vi "Engine_Tick.vi"(0 "Channels":T3, 5 "State":T1={"Tick"=0, "Phase"=0, "PhaseTicks"=0, "Level"=1, "Room"=0, "X10"=0, "Y10"=0, "VY10"=0, "Mode"=0, "Facing"=0, "Run"=0, "Vert"=0, "StandY"=0, "EntryX10"=0, "EntryY10"=0, "EntryMode"=0, "Lives"=4, "Score"=0, "NextLife"=10000, "KeyR"=0, "KeyB"=0, "KeyY"=0, "Torch"=FALSE, "FloorPhase"=0, "Dead"=FALSE, "LevelStart"=FALSE, "Quit"=FALSE, "Sound"=0, "Seed"=12345, "DemoStep"=0, "Tiles"=[], "World"=[], "Enemies"=[], "Highscores"=[], "Name"=[0, 0, 0], "Cursor"=0}, 7 "Rooms":T2(array[cluster]), 11 "error in":errorcluster) -> (4 "State out":T1={"Tick"=0, "Phase"=0, "PhaseTicks"=0, "Level"=1, "Room"=0, "X10"=0, "Y10"=0, "VY10"=0, "Mode"=0, "Facing"=0, "Run"=0, "Vert"=0, "StandY"=0, "EntryX10"=0, "EntryY10"=0, "EntryMode"=0, "Lives"=4, "Score"=0, "NextLife"=10000, "KeyR"=0, "KeyB"=0, "KeyY"=0, "Torch"=FALSE, "FloorPhase"=0, "Dead"=FALSE, "LevelStart"=FALSE, "Quit"=FALSE, "Sound"=0, "Seed"=12345, "DemoStep"=0, "Tiles"=[], "World"=[], "Enemies"=[], "Highscores"=[], "Name"=[0, 0, 0], "Cursor"=0}, 6 "Stop":bool, 15 "error out":errorcluster)   [LabVIEW 2020, in "GH_App.lvlib"]
doc: "One game tick: takes at most one key from the queue, runs Game_Step, sends the sound bits to the audio loop and the new state to the picture loop. Stop on Quit or on an error."
uses:
  GH_App.lvlib
  Engine/GH_Engine.lvlib
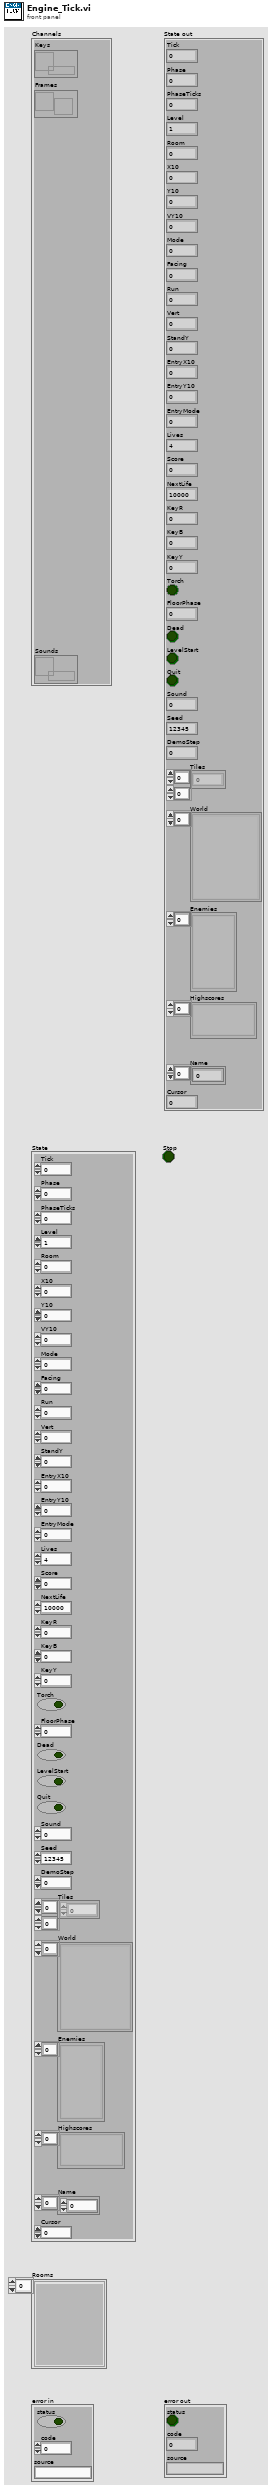
[diagram p1: front panel]
types:
  T1 = cluster{"Tick":u32, "Phase":i32, "PhaseTicks":i32, "Level":i32, "Room":i32, "X10":i32, "Y10":i32, "VY10":i32, "Mode":i32, "Facing":i32, "Run":i32, "Vert":i32, "StandY":i32, "EntryX10":i32, "EntryY10":i32, "EntryMode":i32, "Lives":i32, "Score":i32, "NextLife":i32, "KeyR":i32, "KeyB":i32, "KeyY":i32, "Torch":bool, "FloorPhase":i32, "Dead":bool, "LevelStart":bool, "Quit":bool, "Sound":i32, "Seed":u32, "DemoStep":i32, "Tiles":u8[][], "World":cluster{"ID":string, "Depth":i32, "Column":i32, "Tiles":u8[][]}[], "Enemies":cluster{"Kind":i32, "X10":i32, "Y10":i32, "Dir":i32, "Mode":i32}[], "Highscores":cluster{"Score":i32, "Name":string}[], "Name":i32[], "Cursor":i32}
  T2 = cluster{"ID":string, "Depth":i32, "Column":i32, "Tiles":u8[][]}[]
  T3 = cluster{"Keys":refnum<queue>, "Frames":refnum<notifier>, "Sounds":refnum<queue>}
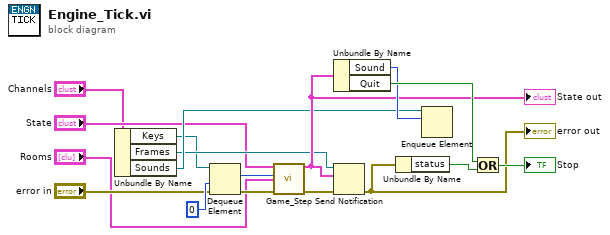
[diagram p0: block diagram]
diagram:
  n1 = Unbundle By Name("Channels") -> ("Keys"=w5:refnum<queue>, "Frames"=w6:refnum<notifier>, "Sounds"=w7:refnum<queue>)
  n2 = Dequeue Element(queue=w5, timeout in ms (-1)=0 ("do not wait"), error in (no error)="error in") -> (element=w9:u16, error out=w10:errorcluster)  [unwired: 2 out]
  n3 = call "Game_Step.vi"("State"="State", "Key"=w9, "Rooms"="Rooms", "error in"=w10) -> ("State out"=w11:T1, "error out"=w12:errorcluster)  [unwired: 10 in]
  "State out" <- w11
  n4 = Unbundle By Name(w11) -> ("Sound"=w13:i32, "Quit"=w14:bool)
  n5 = Send Notification(notification=w11, notifier=w6, error in (no error)=w12) -> (error out=w15:errorcluster)  [unwired: 1 out]
  "error out" <- w15
  n6 = Unbundle By Name(w15) -> ("status"=w16:bool)
  n7 = Enqueue Element(queue=w7, element=w13) -> ()  [unwired: 2 in, 3 out]
  n8 = Or(x=w14, y=w16) -> (x .or. y?=→"Stop":bool)
